vi "start helper loop.vi"(8 "错误输入（无错误）":errorcluster, 10 "helper loop data":T1) -> (0 "错误输出":errorcluster)   [LabVIEW 2025, in "XButton.lvlib" / "button3.xctl"]
uses:
  button3.xctl
  helper loop Events.ctl
  move event.ctl
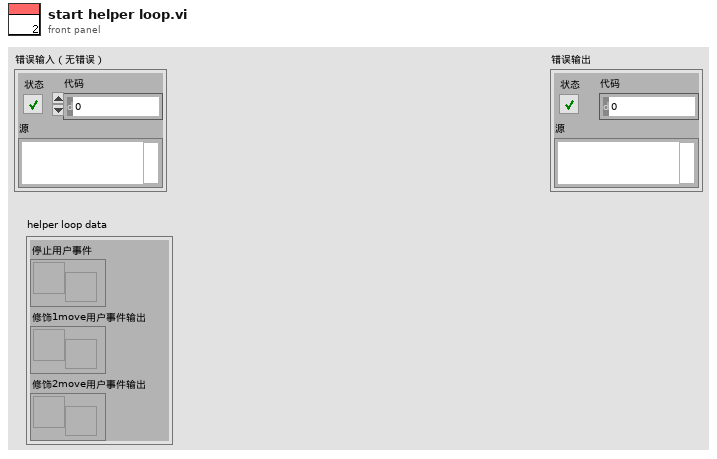
[diagram p1: front panel]
types:
  T1 = typedef "XButton.lvlib/button3.xctl/helper loop Events.ctl" = cluster{"停止用户事件":refnum<user-event>, "修饰1move用户事件输出":refnum<user-event>, "修饰2move用户事件输出":refnum<user-event>}
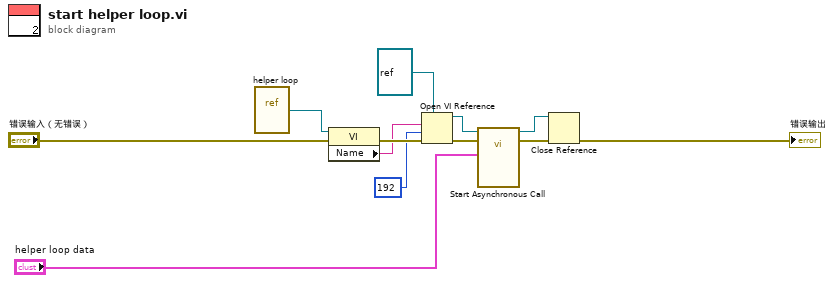
[diagram p0: block diagram]
diagram:
  n1 = vi-ref "helper loop.vi"() -> (w1:refnum<vi>)
  n2 = property class="VI"(reference=w1, error in="错误输入（无错误）") -> (error out=w9:errorcluster, "Name"=w2:string)  [unwired: 1 out]
  n3 = Open VI Reference(type specifier VI Refnum (for type only)=refnum<vi> refnum, vi path=w2, options=192, error in (no error)=w9) -> (vi reference=w5:refnum<vi>, error out=w6:errorcluster)  [unwired: 2 in]
  n4 = call-by-ref "Start Asynchronous Call"(reference=w5, error in=w6, "helper loop data"="helper loop data") -> (reference out=w3:refnum<vi>, error out=w4:errorcluster)  [unwired: 11 in]
  n5 = Close Reference(reference=w3, error in (no error)=w4) -> (error out=→"错误输出":errorcluster)
